vi "Plot menu activation GENERAL.vi"(5 "panel mode":T1, 7 "menu tag":string, 8 "error in (no error)":errorcluster, 11 "MenuRef":refnum<k9>) -> (0 "error out":errorcluster, 3 "MenuRef":refnum<k9>)   [LabVIEW 2021, in "RocketPlot.lvlib"]
uses:
  RocketPlot.lvlib
  TypeDefs/panel mode.ctl
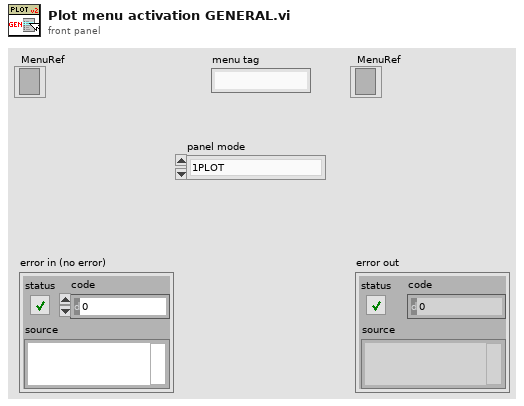
[diagram p1: front panel]
types:
  T1 = typedef "RocketPlot.lvlib/panel mode.ctl" = enum16{"1PLOT", "MPLOT"}
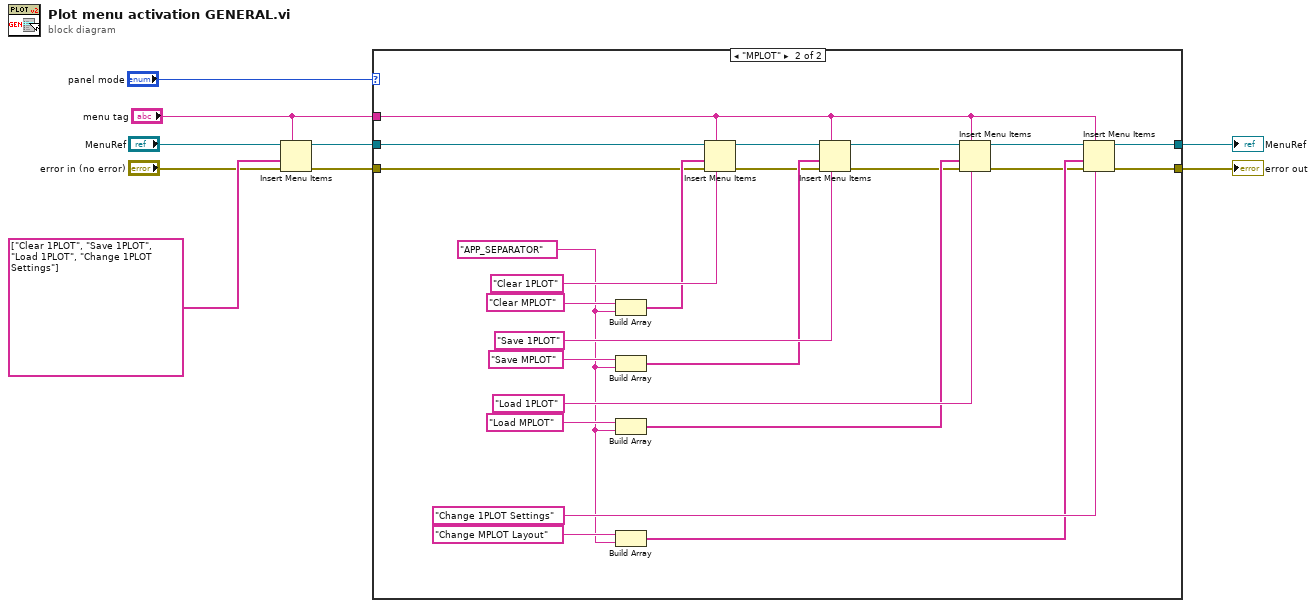
[diagram p0: block diagram]
diagram:
  n1 = Insert Menu Items(5:"menu tag", 6:"error in (no error)", 7:string[] ["Clear 1PLOT", "Save 1PLOT", "Load 1PLOT", "Change 1PLOT Settings"], 9:"MenuRef") -> (0:w3:errorcluster, 3:w5:refnum<k9>)  [unwired: 2 in, 1 out]
  n2 = case shown="\"MPLOT\"" "panel mode" {
    tunnel: w5 -> [w11 w35]
    tunnel: [w11 w19] -> w1
    tunnel: w3 -> [w10 w18]
    tunnel: [w10 w15] -> w2
    tunnel: "menu tag" -> [_ w14]
    frame "1PLOT" {
    }
    frame "MPLOT" {
      w25 = "APP_SEPARATOR"
      n3 = Build Array("Clear MPLOT", w25) -> (w29:string[])
      n4 = Build Array("Save MPLOT", w25) -> (w24:string[])
      n5 = Build Array("Load MPLOT", w25) -> (w23:string[])
      n6 = Build Array("Change MPLOT Layout", w25) -> (w22:string[])
      n7 = Insert Menu Items(4:"Clear 1PLOT", 5:w14, 6:w18, 7:w29, 9:w35) -> (0:w17:errorcluster, 3:w21:refnum<k9>)  [unwired: 1 in, 1 out]
      n8 = Insert Menu Items(4:"Save 1PLOT", 5:w14, 6:w17, 7:w24, 9:w21) -> (0:w16:errorcluster, 3:w20:refnum<k9>)  [unwired: 1 in, 1 out]
      n9 = Insert Menu Items(4:"Load 1PLOT", 5:w14, 6:w16, 7:w23, 9:w20) -> (0:w13:errorcluster, 3:w12:refnum<k9>)  [unwired: 1 in, 1 out]
      n10 = Insert Menu Items(4:"Change 1PLOT Settings", 5:w14, 6:w13, 7:w22, 9:w12) -> (0:w15:errorcluster, 3:w19:refnum<k9>)  [unwired: 1 in, 1 out]
    }
  }
  "error out" <- w2
  "MenuRef" <- w1
